vi "Execute SequenceFile.vi"() -> ()   [LabVIEW 2020]
uses:
  Data Types/File Load Options.ctl
  VariableContainer/Set Value STR.vi
  VariableContainer/Set Value BOOL.vi
  VariableContainer/Set Value U64.vi
  Execution/Set Entry Sequence.vi
  Execution/Set Sequence File.vi
  Execution/Set Parameters.vi
  Execution/Execution.lvclass
  Engine/Engine.lvclass
  VariableContainer/VariableContainer.lvclass
  HTS.lvlib
  VariableContainer/Set Value VAR.vi
panel:
  in  "Terminate":bool
  in  "Resume":bool
  in  "Params":T1={"SerialNo"="ABC123", "TestBool"=TRUE, "DeviceID"=5648432}
  out "error out":errorcluster
  in  "Sequence":string="MainSequence"
  in  "SequenceFile Path":path=path "C:/dev/Negentropic/HTS/Test/Sequences/DisplaySerialNo.seq"
  # "The sequence will pause immediately when starting, choose resume to run it and get the dialog or terminate to cancel execution."
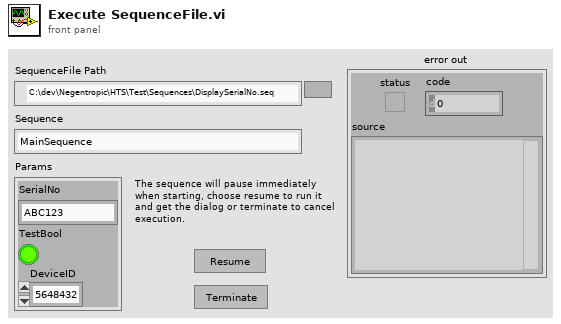
[diagram p1: front panel]
types:
  T1 = cluster{"SerialNo":string, "TestBool":bool, "DeviceID":u64}
  T2 = typedef "HTS.lvlib/File Load Options.ctl" = cluster{"Use Search Dirs? (T)":bool, "Conflict as Error? (T)":bool, "Check Station Model? (F)":bool, "Preload Modules? (T)":bool, "Skip Load Callback? (F)":bool, "Reload if Loaded? (F)":bool}
  T3 = typedef "HTS.lvlib/Engine.lvclass/Session Handle.ctl" = refnum<data-value>
  T4 = typedef "HTS.lvlib/SequenceFile.lvclass/Session Handle.ctl" = refnum<data-value>
  T5 = typedef "HTS.lvlib/Execution.lvclass/Session Handle.ctl" = refnum<data-value>
  T6 = typedef "HTS.lvlib/VariableContainer.lvclass/Session Handle.ctl" = refnum<data-value>
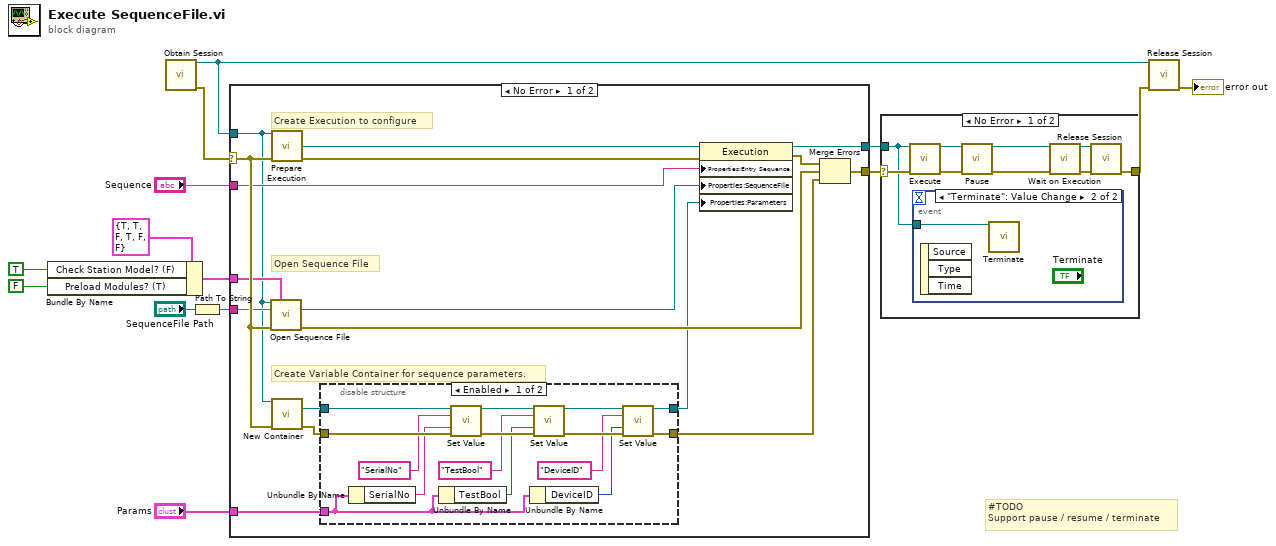
[diagram p0: block diagram]
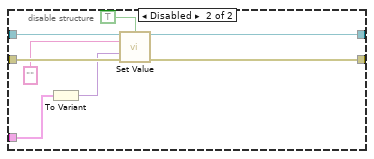
[diagram p2: hidden frame]
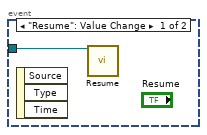
[diagram p4: hidden frame]
diagram:
  # "#TODO\nSupport pause / resume / terminate"
  n1 = Bundle By Name(cluster=T2 {"Use Search Dirs? (T)"=TRUE, "Conflict as Error? (T)"=TRUE, "Check Station Model? (F)"=FALSE, "Preload Modules? (T)"=TRUE, "Skip Load Callback? (F)"=FALSE, "Reload if Loaded? (F)"=FALSE} ("Load Options"), "Check Station Model? (F)"=TRUE, "Preload Modules? (T)"=FALSE) -> (w7:T2)
  n2 = call "Obtain Session.vi"() -> ("Session Handle"=w4:T3, "error out"=w5:errorcluster)  [unwired: 14 in]
  n3 = Path To String(path="SequenceFile Path") -> (string=w6:string)
  n4 = case shown="No Error" w5 {
    selector: w5 -> [w31 w55]
    tunnel: [w25 _] -> w1
    tunnel: "Sequence" -> [w18 _]
    tunnel: w7 -> [w20 _]
    tunnel: w6 -> [w19 _]
    tunnel: [w22 w55] -> w2
    tunnel: w4 -> [w16 _]
    tunnel: "Params" -> [w17 _]
    frame No Error {
      # "Create Variable Container for sequence parameters."
      # "Open Sequence File"
      # "Create Execution to configure"
      n5 = call "Open Sequence File.vi"("Session Handle in"=w16, "Load Options"=w20, "File Path"=w19, "error in (no error)"=w31) -> ("SequenceFile"=w26:T4, "error out"=w29:errorcluster)  [unwired: 9 in, 1 out]
      n6 = call "Prepare Execution.vi"("Session Handle in"=w16, "error in (no error)"=w31) -> ("Execution"=w21:T5, "error out"=w24:errorcluster)  [unwired: 11 in, 1 out]
      n7 = call "New Container.vi"("Session Handle in"=w16, "error in (no error)"=w31) -> ("New Value Container"=w27:T6, "error out"=w28:errorcluster)  [unwired: 11 in, 1 out]
      n8 = disable-structure shown="Enabled" {
        disable-tunnel: [w46 w50] -> w30
        disable-tunnel: w28 -> [w45 w53]
        disable-tunnel: w27 -> [w37 w54]
        disable-tunnel: [w36 w49] -> w15
        disable-tunnel: w17 -> [w32 w51]
        frame Enabled {
          n9 = Unbundle By Name(w32) -> ("SerialNo"=w35:string)
          n10 = Unbundle By Name(w32) -> ("TestBool"=w34:bool)
          n11 = call-poly "Set Value.vi"("Session Handle in"=w37, "Lookup String"="SerialNo", "Value"=w35, "error in (no error)"=w45) -> ("Session Handle out"=w41:T6, "error out"=w43:errorcluster)  [unwired: 10 in]
          n12 = Unbundle By Name(w32) -> ("DeviceID"=w33:u64)
          n13 = call-poly "Set Value.vi"("Session Handle in"=w41, "Lookup String"="TestBool", "Value"=w34, "error in (no error)"=w43) -> ("Session Handle out"=w39:T6, "error out"=w44:errorcluster)  [unwired: 10 in]
          n14 = call-poly "Set Value.vi"("Session Handle in"=w39, "Lookup String"="DeviceID", "Value"=w33, "error in (no error)"=w44) -> ("Session Handle out"=w36:T6, "error out"=w46:errorcluster)  [unwired: 10 in]
        }
        frame Disabled {
          n15 = To Variant(anything=w51) -> (Variant=w48:variant)
          n16 = call-poly "Set Value.vi"("Session Handle in"=w54, "Skip Outer Cluster (T)"=TRUE, "Lookup String"="", "Value"=w48, "error in (no error)"=w53) -> ("Session Handle out"=w49:T6, "error out"=w50:errorcluster)  [unwired: 9 in]
        }
      }
      n17 = property class="Execution"(reference=w21, error in=w24, "Properties:Entry Sequence"=w18, "Properties:SequenceFile"=w26, "Properties:Parameters"=w15) -> (reference out=w25:T5, error out=w23:errorcluster)
      n18 = Merge Errors(w23, w29, w30) -> (w22:errorcluster)
    }
    frame Error {
    }
  }
  n19 = case shown="No Error" w2 {
    selector: w2 -> [w64 w67]
    tunnel: w1 -> [w56 _]
    tunnel: [w61 w67] -> w12
    frame No Error {
      n20 = call "Execute.vi"("Session Handle in"=w56, "error in (no error)"=w64) -> ("Session Handle out"=w60:T5, "error out"=w59:errorcluster)  [unwired: 12 in]
      n21 = event shown="[1] \"Terminate\": Value Change" {
        selector: _ -> [_ _]
        dyn-events: _ -> [_ _]
        timeout: _ -> [_ _]
        tunnel: w56 -> [w65 w66]
        event "Resume": Value Change {
          n22 = event-data() -> ()  [unwired: 1 in, 3 out]
          n23 = call "Resume.vi"("Session Handle in"=w65) -> ()  [unwired: 13 in, 2 out]
        }
        event "Terminate": Value Change {
          n24 = event-data() -> ()  [unwired: 1 in, 3 out]
          n25 = call "Terminate.vi"("Session Handle in"=w66) -> ()  [unwired: 13 in, 2 out]
        }
      }
      n26 = call "Pause.vi"("Session Handle in"=w60, "error in (no error)"=w59) -> ("Session Handle out"=w57:T5, "error out"=w58:errorcluster)  [unwired: 12 in]
      n27 = call "Wait on Execution.vi"("Session Handle in"=w57, "error in (no error)"=w58) -> ("Session Handle out"=w62:T5, "error out"=w63:errorcluster)  [unwired: 11 in, 1 out]
      n28 = call "Release Session.vi"("Session Handle"=w62, "error in (no error)"=w63) -> ("error out"=w61:errorcluster)  [unwired: 13 in]
    }
    frame Error {
    }
  }
  n29 = call "Release Session.vi"("Session Handle"=w4, "error in (no error)"=w12) -> ("error out"=→"error out":errorcluster)  [unwired: 13 in]
